vi "Sensor Pos to Trap Pos.vi"(11 "Sensor Pos":dbl) -> (3 "Trapezoid Pos":dbl)   [LabVIEW 2027]
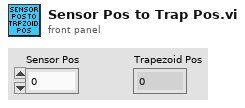
[diagram p1: front panel]
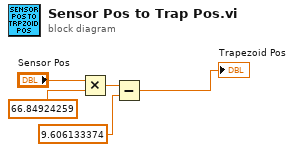
[diagram p0: block diagram]
diagram:
  n1 = Multiply(x="Sensor Pos", y=66.84924259) -> (x*y=w3:dbl)
  n2 = Subtract(x=w3, y=9.606133374) -> (x-y=→"Trapezoid Pos":dbl)
